vi "Logger_Init.vi"(8 "error in (no error)":errorcluster, 11 "base path":path) -> (0 "error out":errorcluster, 2 "state":T1, 3 "Folder ready":path)   [LabVIEW 2025]
uses:
  Logger_State.ctl
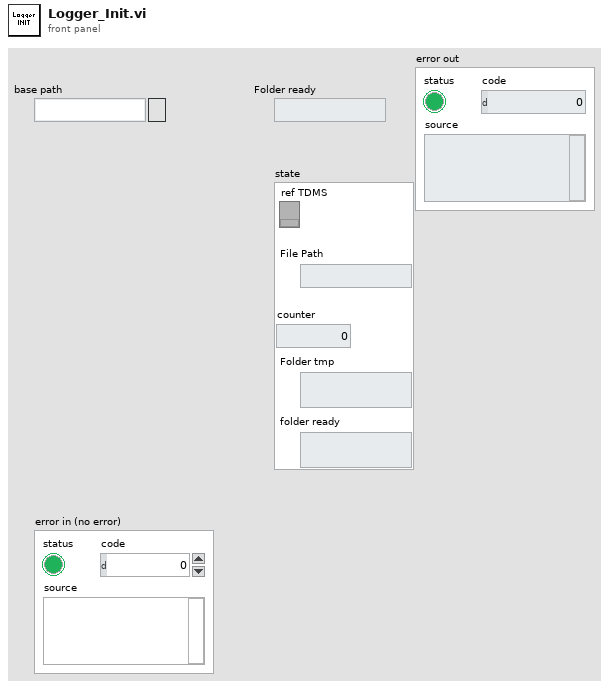
[diagram p1: front panel]
types:
  T1 = typedef "Logger_State.ctl" = cluster{"ref TDMS":refnum<k34>, "File Path":path, "counter":i32, "Folder tmp":path, "folder ready":path}
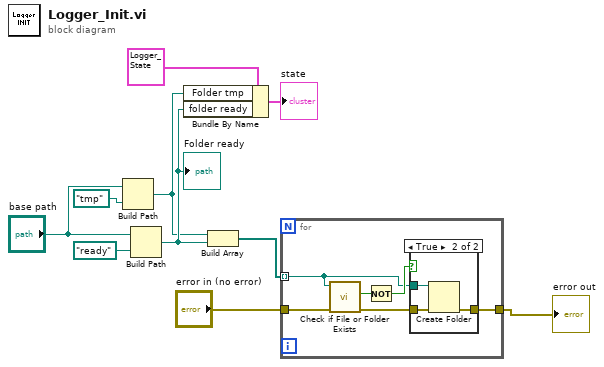
[diagram p0: block diagram]
diagram:
  n1 = Build Path(base path="base path", name or relative path=path "tmp") -> (appended path=w8:path)
  n2 = Build Path(base path="base path", name or relative path=path "ready") -> (appended path=w10:path)
  "Folder ready" <- w10
  n3 = Bundle By Name(cluster=T1 {"ref TDMS"=refnum, "File Path"=path "", "counter"=0, "Folder tmp"=path "/home/lvuser/lab9data/tmp", "folder ready"=path "/home/lvuser/lab9data/ready"} ("Logger_state"), "Folder tmp"=w8, "folder ready"=w10) -> (→"state":T1)
  n4 = Build Array(w8, w10) -> (w5:path[])
  n5 = for {
    tunnel: w5 -> [w14] mode=indexing
    tunnel: "error in (no error)" -> [w13]
    tunnel: [w11] -> w1
    n6 = call <vilib>:"Check if File or Folder Exists.vi"("error in (no error)"=w13, "path"=w14) -> ("error out"=w12:errorcluster, "file or folder exists?"=w16:bool)  [unwired: 7 in, 1 out]
    n7 = Not(x=w16) -> (.not. x?=w15:bool)
    n8 = case shown="True" w15 {
      tunnel: w14 -> [_ w20]
      tunnel: w12 -> [w17 w19]
      tunnel: [w17 w18] -> w11
      frame False {
      }
      frame True {
        n9 = Create Folder(path (use dialog)=w20, error in=w19) -> (error out=w18:errorcluster)  [unwired: 1 in, 2 out]
      }
    }
  }
  "error out" <- w1
